vi "Step_Begin.vi"(8 "error in (no error)":errorcluster={"status"=FALSE, "code"=0, "source"="\"\""}, 10 "active run/cycle refs":string, 11 "ActionDefinition":string) -> (0 "error out":errorcluster={"status"=FALSE, "code"=0, "source"="\"\""}, 2 "status ok":bool, 3 "StepContext":string)   [LabVIEW 2026]
doc: "INTENT: Create action instance. LOGIC: Set status active, phase precheck, assign action instance ID, deadlines and capture policy."
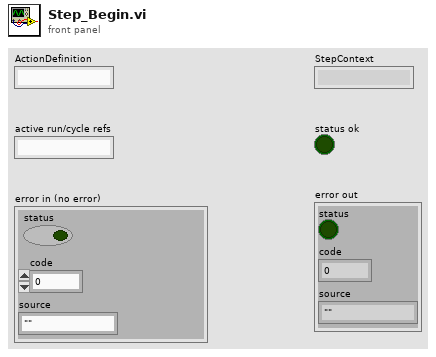
[diagram p1: front panel]
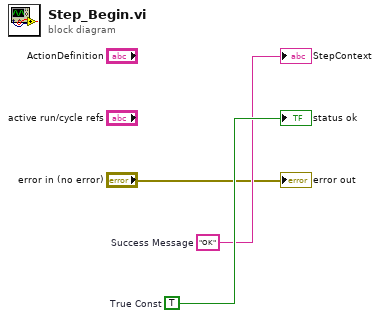
[diagram p0: block diagram]
diagram:
  w3 = TRUE  # True Const
  w2 = "OK"  # Success Message
  "StepContext" <- w2
  "status ok" <- w3
  "error out" <- "error in (no error)"
